vi "ASM MIni Stat.vi"(6 "error in":errorcluster, 8 "Base Table":T2(array[cluster]) {"Value 3" format="%.2g"}, 10 "Sample Sequence":string="TGTXCT", 11 "Right Read MIN":i32=4) -> (0 "SB_ANA":T1, 3 "RR Ratio (%)":dbl format="%.3g", 4 "error out":errorcluster)   [LabVIEW 2018]
panel:
  out "Base Species#":i32
  out "all option#":i32
  out "Potential Canditate#":i32[](array[numeric])
  out "RRS#":i32
  out "RR Seq":T3
  out "Base Cutted Q#":i32
  out "RR option#":i32
  out "Cutted Sequence":string
  out "サイズ":i32
  out "RR Canditate#":i32[](array[numeric])
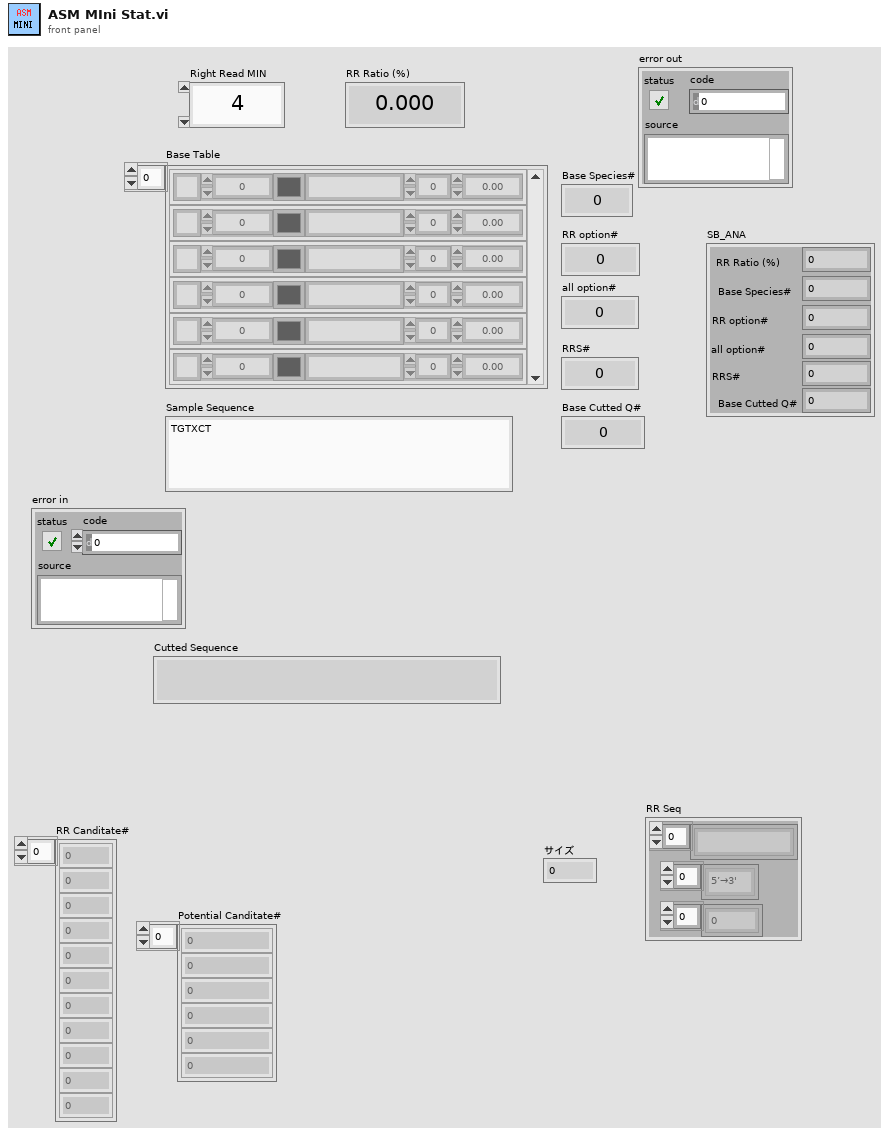
[diagram p1: front panel]
types:
  T1 = cluster{"RR Ratio (%)":dbl, "Base Species#":i32, "RR option#":i32, "all option#":i32, "RRS#":i32, "Base Cutted Q#":i32}
  T2 = cluster{"Name":string, "Value":dbl, "Color":u32, "Name 2":string, "Value 2":dbl, "Value 3":dbl}[]
  T3 = cluster{string[], enum16{"5’→3'", "3'→5'"}[], i32[]}
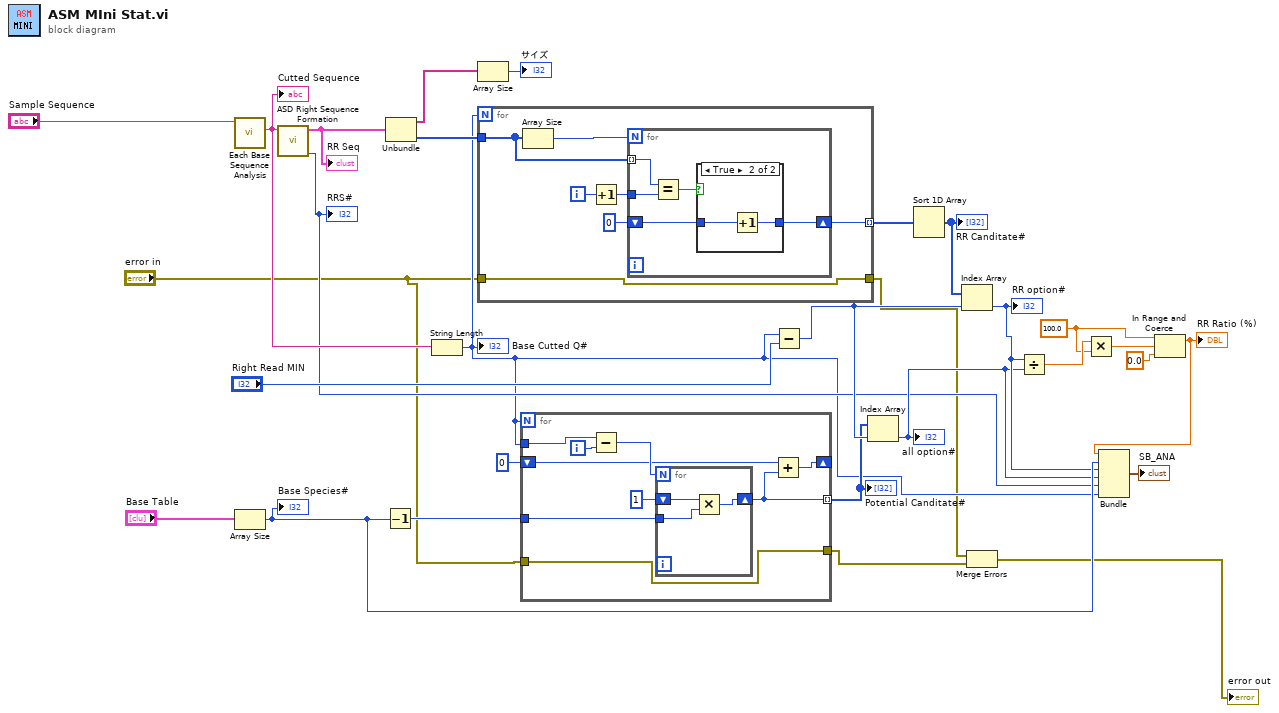
[diagram p0: block diagram]
diagram:
  w15 = 100.0 ("y")
  n1 = call "Each Base Sequence Analysis.vi"("Sample Sequence"="Sample Sequence") -> ("Cutted Sequence"=w27:string)  [unwired: 7 in, 3 out]
  "Cutted Sequence" <- w27
  n2 = Array Size(array="Base Table") -> (size(s)=w11:i32)
  "Base Species#" <- w11
  n3 = call "ASD Right Sequence Formation.vi"("Sample Sequence"=w27) -> ("RRS#"=w8:i32, "RR Seq"=w23:T3)  [unwired: 9 in]
  "RRS#" <- w8
  "RR Seq" <- w23
  n4 = Decrement(x=w11) -> (x-1=w26:i32)
  n5 = Unbundle(w23) -> (w21:string[], w20:i32[])  [unwired: 1 out]
  n6 = String Length(string=w27) -> (length=w7:i32)
  "Base Cutted Q#" <- w7
  n7 = Array Size(array=w21) -> (size(s)=→"サイズ":i32)
  n8 = for {
    N: w7 -> [_]
    tunnel: w20 -> [w36]
    tunnel: [w33] -> w19 mode=indexing
    tunnel: "error in" -> [w30]
    tunnel: [w30] -> w3
    i -> [w32]
    n9 = Array Size(array=w36) -> (size(s)=w35:i32)
    n10 = Increment(x=w32) -> (x+1=w31:i32)
    n11 = for {
      N: w35 -> [_]
      tunnel: w36 -> [w41] mode=indexing
      shift-right: [w39] -> w33
      shift-left: 0 -> [w38]
      tunnel: w31 -> [w37]
      n12 = Equal?(x=w41, y=w37) -> (x = y?=w40:bool)
      n13 = case shown="True" w40 {
        tunnel: [w42 w44] -> w39
        tunnel: w38 -> [w42 w43]
        frame False {
        }
        frame True {
          n14 = Increment(x=w43) -> (x+1=w44:i32)
        }
      }
    }
  }
  n15 = for {
    N: w7 -> [_]
    tunnel: w7 -> [w50]
    tunnel: w26 -> [w53]
    shift-right: [w47] -> _
    shift-left: 0 -> [w48]
    tunnel: [w46] -> w12 mode=indexing
    tunnel: "error in" -> [w45]
    tunnel: [w45] -> w2
    i -> [w49]
    n16 = Subtract(x=w50, y=w49) -> (x-y=w51:i32)
    n17 = for {
      N: w51 -> [_]
      tunnel: w53 -> [w56]
      shift-right: [w55] -> w46
      shift-left: 1 -> [w54]
      n18 = Multiply(x=w54, y=w56) -> (x*y=w55:i32)
    }
    n19 = Add(x=w48, y=w46) -> (x+y=w47:i32)
  }
  "Potential Canditate#" <- w12
  n20 = Subtract(x=w7, y="Right Read MIN") -> (x-y=w17:i32)
  n21 = Index Array(array=w12, index=w17) -> (element=w9:i32)
  "all option#" <- w9
  n22 = Sort 1D Array(array=w19) -> (sorted array=w13:i32[])
  "RR Canditate#" <- w13
  n23 = Index Array(array=w13, index=w17) -> (element=w10:i32)
  "RR option#" <- w10
  n24 = Merge Errors(w3, w2) -> (→"error out":errorcluster)
  n25 = Divide(x=w10, y=w9) -> (x/y=w24:dbl)
  n26 = Multiply(x=w24, y=w15) -> (x*y=w16:dbl)
  n27 = In Range and Coerce(upper limit=w15, x=w16, lower limit=0.0 ("下限")) -> (coerced(x)=w6:dbl)  [unwired: 1 out]
  "RR Ratio (%)" <- w6
  n28 = Bundle("y"=w6, w11, w10, w9, "RRS#"=w8, w7) -> (→"SB_ANA":cluster{"y":dbl, i32, i32, i32, "RRS#":i32, i32})  [unwired: 1 in]
